vi "variant to u32.vi"(1 "Variant":variant) -> (0 "U32":u32)   [LabVIEW 2025]
doc: "convert variant data to a LabVIEW 4-Byte unsigned Integer (U32)\n<B>Input:</B>\nVariant (skalar)\n<B>Output:</B>\n4-Byte unsigned Integer (U32)"
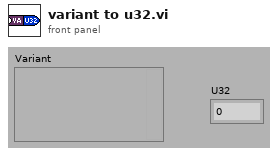
[diagram p1: front panel]
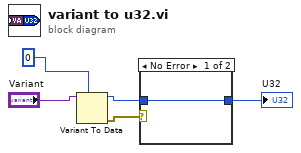
[diagram p0: block diagram]
diagram:
  n1 = Variant To Data(type=u32 0 ("MIN U/36V"), Variant="Variant") -> (data=w4:u32, error out=w3:errorcluster)  [unwired: 1 in]
  n2 = case shown="No Error" w3 {
    tunnel: w4 -> [w6 _]
    tunnel: [w6 _] -> w5
    frame No Error {
    }
    frame Error {
    }
  }
  "U32" <- w5
